vi "Get Current User.vi"(4 "error in (no error)":errorcluster, 7 "EasyUserManager in":refnum<class "EasyUserManager.lvclass">) -> (0 "error out":errorcluster, 2 "LoginName":string, 3 "EasyUserManager out":refnum<class "EasyUserManager.lvclass">)   [LabVIEW 2024, in "EasyUserManager.lvclass"]
doc: "This VI returns the <b>LoginName</b> of the currently logged in user."
uses:
  EasyUserManager.lvclass
  EasyUserManager.lvclass/EasyUserManager.ctl
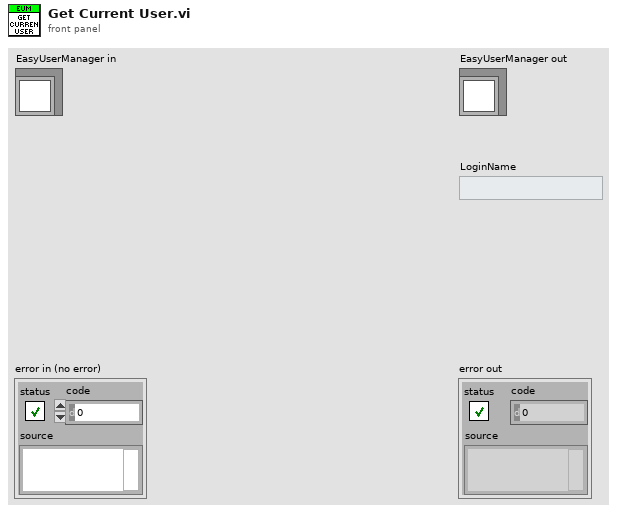
[diagram p1: front panel]
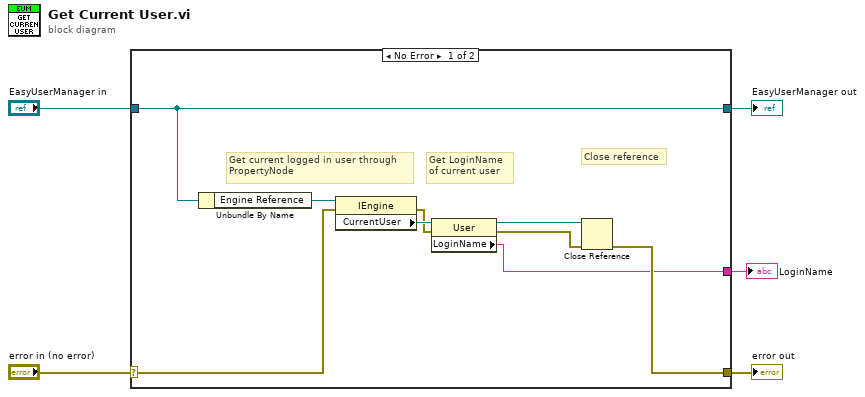
[diagram p0: block diagram]
diagram:
  n1 = case shown="No Error" "error in (no error)" {
    selector: "error in (no error)" -> [w12 w16]
    tunnel: [w7 w16] -> w4
    tunnel: [w14 w15] -> w2
    tunnel: "EasyUserManager in" -> [w14 w15]
    tunnel: [w6 _] -> w1
    frame No Error {
      # "Close reference"
      # "Get LoginName\nof current user"
      # "Get current logged in user through\nPropertyNode"
      n2 = Unbundle By Name(w14) -> ("Engine Reference"=w13:refnum<k7>)
      n3 = property on="Property Node" class="IEngine"(reference=w13, error in=w12) -> (error out=w10:errorcluster, "CurrentUser"=w11:refnum<k7>)  [unwired: 1 out]
      n4 = property on="Property Node" class="User"(reference=w11, error in=w10) -> (reference out=w9:refnum<k7>, error out=w8:errorcluster, "LoginName"=w6:string)
      n5 = Close Reference(reference=w9, error in (no error)=w8) -> (error out=w7:errorcluster)
    }
    frame Error {
      # "Pass error and do nothing."
    }
  }
  "error out" <- w4
  "EasyUserManager out" <- w2
  "LoginName" <- w1
